vi "Write Sensor Loop Rate.vi"(10 "Sensor Loop Rate":dbl, 11 "LabjacksController in":refnum<class "LabjacksController.lvclass">) -> (3 "LabjacksController out":refnum<class "LabjacksController.lvclass">)   [LabVIEW 2025, in "LabjacksController.lvclass"]
uses:
  LabjacksController.lvclass
  LabjacksController.lvclass/LabjacksController.ctl
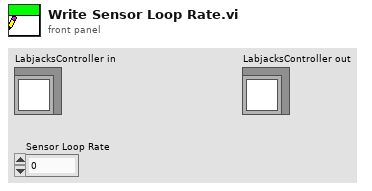
[diagram p1: front panel]
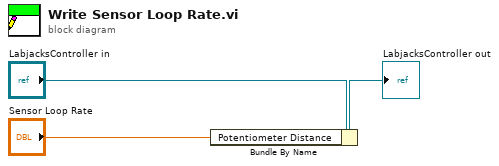
[diagram p0: block diagram]
diagram:
  n1 = Bundle By Name(cluster="LabjacksController in", "Potentiometer Distance"="Sensor Loop Rate") -> (→"LabjacksController out":refnum<class "LabjacksController.lvclass">)
